vi "Send Get Input.vi"(7 "Message Priority (Normal)":T1=enum."Normal", 8 "error in (no error)":errorcluster, 10 "DIO_CFG":refnum<class "DIO-Configuration.lvclass">, 11 "Message Enqueuer":refnum<class "Message Enqueuer.lvclass">) -> (0 "error out":errorcluster, 2 "Input":bool, 3 "Message Enqueuer out":refnum<class "Message Enqueuer.lvclass">)   [LabVIEW 2021, in "Simulator-Channel.lvlib" / "DIO_Panel.lvlib" / "Get Input Msg.lvclass"]
doc: "This VI sends the message to an actor."
uses:
  Get Input Msg.lvclass
  <vilib>/ActorFramework/Message Enqueuer/Message Enqueuer.lvclass
  <vilib>/ActorFramework/Message Enqueuer/Message Priority.ctl
  Dependencies/DIO-Channel.lvlibp/Channels/DIO-Channel/DIO-Configuration_class/DIO-Configuration.lvclass
  C:/Program Files/National Instruments/LabVIEW 2021/vi.lib/ActorFramework/Message/Message.lvclass
  Get Input Msg.lvclass/Get Input Msg.ctl
  <vilib>/ActorFramework/Message Enqueuer/Message Enqueuer.lvclass/Message Enqueuer.ctl
  <vilib>/ActorFramework/Message Priority Queue/Priority Enqueue.vi
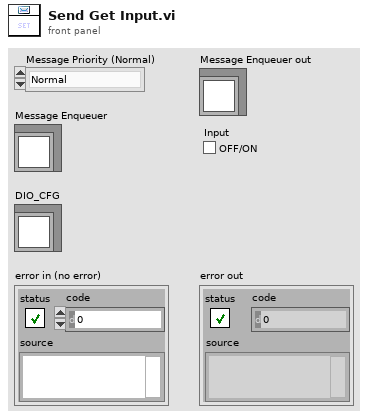
[diagram p1: front panel]
types:
  T1 = typedef "Actor Framework.lvlib/Message Enqueuer.lvclass/Message Priority.ctl" = enum16{"Low", "Normal", "High"}
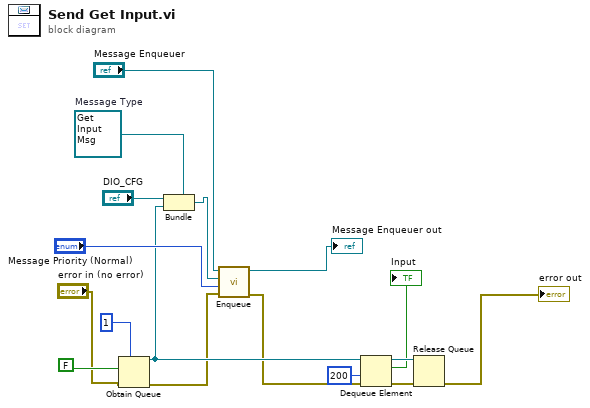
[diagram p0: block diagram]
diagram:
  w17 = refnum<class "Get Input Msg.lvclass"> refnum  # Message Type
  n1 = Obtain Queue(max queue size (-1, unlimited)=1, element data type=FALSE, error in (no error)="error in (no error)") -> (queue out=w6:refnum<queue>, error out=w2:errorcluster)  [unwired: 2 in, 1 out]
  n2 = Bundle(cluster=w17, "DIO_CFG", w6) -> (w12:refnum<class "Get Input Msg.lvclass">)
  n3 = call <vilib>:"Enqueue.vi"("error in (no error)"=w2, "Message Priority (Normal)"="Message Priority (Normal)", "Message"=w12, "Message Enqueuer in"="Message Enqueuer") -> ("error out"=w4:errorcluster, "Message Enqueuer out"=→"Message Enqueuer out":refnum<class "Message Enqueuer.lvclass">)  [unwired: 6 in]
  n4 = Dequeue Element(queue=w6, timeout in ms (-1)=200, error in (no error)=w4) -> (queue out=w8:refnum<queue>, element=→"Input":bool, error out=w7:errorcluster)  [unwired: 1 out]
  n5 = Release Queue(queue=w8, error in (no error)=w7) -> (error out=→"error out":errorcluster)  [unwired: 1 in, 2 out]
